vi "RDV-handle-AllPermTypes.vi"(8 "error in (no error)":errorcluster, 11 "RDV-Reflection_Data_viewer in":refnum<class "RDV-Reflection_Data_viewer.lvclass">) -> (0 "error out":errorcluster, 3 "RDV-Reflection_Data_viewer out":refnum<class "RDV-Reflection_Data_viewer.lvclass">)   [LabVIEW 2020, in "RDV-Reflection_Data_viewer.lvclass"]
doc: "Computes the permittivity of all data in the viewer's map with every calculation method, using RDC-permittivity-handle_matrix, and adds the results to the map."
uses:
  RDV-Reflection_Data_viewer.lvclass
  RDV-Reflection_Data_viewer.lvclass/RDV-Reflection_Data_viewer.ctl
  Computation/RDC-Reflection_Data_Computation.lvlib
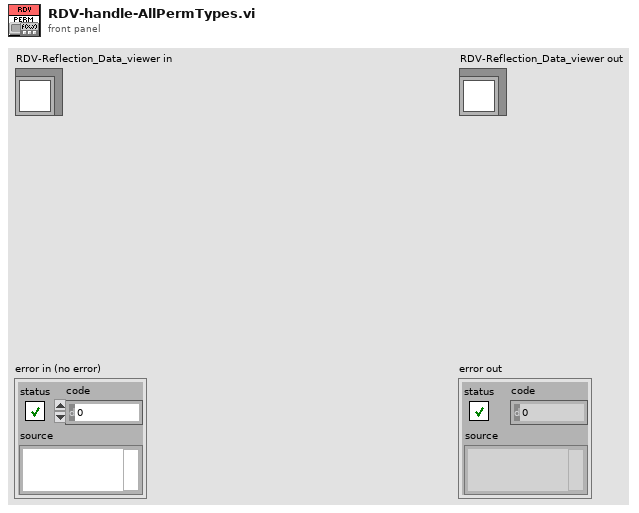
[diagram p1: front panel]
types:
  T1 = typedef "RDV-Reflection_Data_viewer.lvclass/RDV-UPDATE_IGNORE_LIST.ctl" = string[]
  T2 = typedef "RFH-Reflection_File_Handler.lvlib/RFH-common_data_format.ctl" = cluster{"Frequency":dbl[], "Reflection'":dbl[], "Reflection''":dbl[], "Permativity'":dbl[], "Permativity''":dbl[], "Conductivity":dbl[], "Loss Tangent":dbl[], "Resistance":dbl[], "Reactance":dbl[]}
  T3 = typedef "RDV-Reflection_Data_viewer.lvclass/RDV-DATA_MAP_CLUST.ctl" = cluster{"filename w/ ext":string, "Common Format":T2}
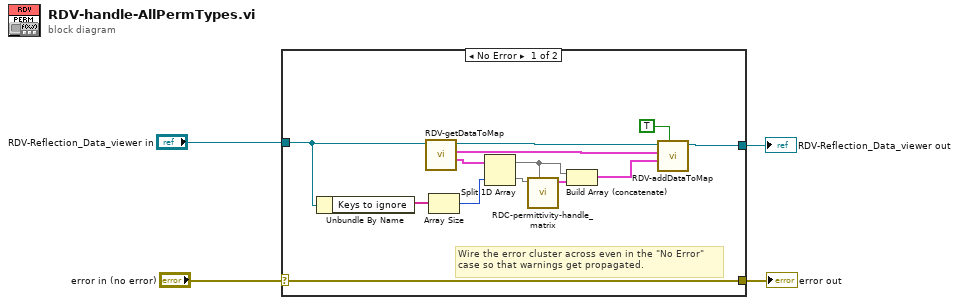
[diagram p0: block diagram]
diagram:
  n1 = case shown="No Error" "error in (no error)" {
    selector: "error in (no error)" -> [w17 w19]
    tunnel: [w17 w19] -> w3
    tunnel: [w5 w18] -> w1
    tunnel: "RDV-Reflection_Data_viewer in" -> [w16 w18]
    frame No Error {
      # "Wire the error cluster across even in the \"No Error\"\ncase so that warnings get propagated."
      n2 = Unbundle By Name(w16) -> ("Keys to ignore"=w15:T1)
      n3 = call "RDV-getDataToMap.vi"("RDV-Reflection_Data_viewer in"=w16) -> ("data"=w13:T2[], "all data"=w11:cluster{"key":string, "data":T3}[], "RDV-Reflection_Data_viewer out"=w12:refnum<class "RDV-Reflection_Data_viewer.lvclass">)  [unwired: 7 in, 1 out]
      n4 = Array Size(array=w15) -> (size(s)=w14:i32)
      n5 = Split 1D Array(array=w13, index=w14) -> (first subarray=w10:T2[], second subarray=w9:T2[])
      n6 = call "RDC-permittivity-handle_matrix.vi"("basic data(open, short, water, ...)"=w10, "Data Array"=w9) -> ("Common Format out"=w6:T2[])  [unwired: 9 in]
      n7 = Build Array (concatenate)(w10, w6) -> (w8:T2[])
      n8 = call "RDV-addDataToMap.vi"("Use ignore list (false)"=TRUE, "data"=w8, "all data"=w11, "RDV-Reflection_Data_viewer in"=w12) -> ("RDV-Reflection_Data_viewer out"=w5:refnum<class "RDV-Reflection_Data_viewer.lvclass">)  [unwired: 6 in, 1 out]
    }
    frame Error {
    }
  }
  "error out" <- w3
  "RDV-Reflection_Data_viewer out" <- w1
